vi "Wait For Stream Drain.vi"(8 "error in":errorcluster, 10 "timeout ms":i32=1000, 11 "events":refnum<queue>) -> (0 "error out":errorcluster, 3 "drained?":bool)   [LabVIEW 2020, in "MCP Server.lvlib"]
doc: "Waits until the events queue of a streamed tools/call is empty, polling every 20 ms, for at most timeout ms.\n\nWhile the client is connected, the IG HTTP Server sends one event per Next Segment call and asks for the next one straight away, so the queue empties within milliseconds. When the client has closed the stream, a chunk write fails, the server stops asking and nothing empties the queue any more: drained? stays FALSE. That is how a closed stream (the MCP cancellation signal over HTTP) is noticed. An invalid or released queue also gives FALSE."
uses:
  MCP Server.lvlib
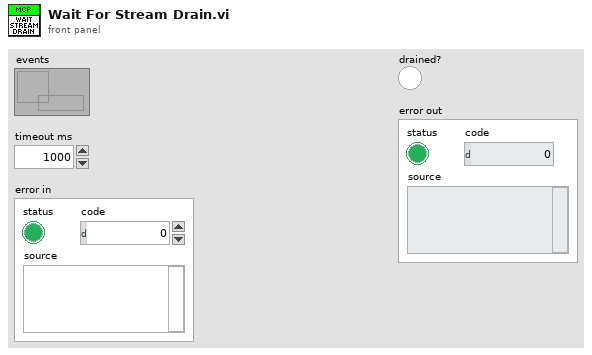
[diagram p1: front panel]
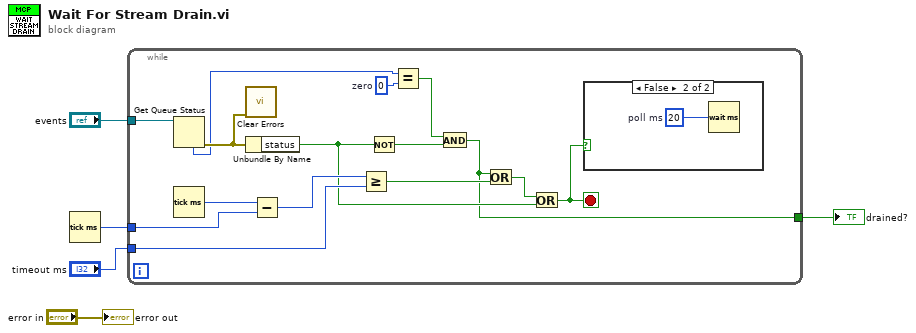
[diagram p0: block diagram]
diagram:
  n1 = Tick Count (ms)() -> (millisecond timer value=w4:u32)
  n2 = while {
    tunnel: "events" -> [w20]
    tunnel: w4 -> [w13]
    tunnel: "timeout ms" -> [w11]
    tunnel: [w6] -> w2
    stop <- w7 stop-if-true
    w17 = 0  # zero
    n3 = Get Queue Status(queue=w20) -> (error out=w19:errorcluster, # elements in queue=w18:i32)  [unwired: 2 in, 6 out]
    n4 = Tick Count (ms)() -> (millisecond timer value=w14:u32)
    n5 = call <vilib>:"Clear Errors.vi"("error in (no error)"=w19) -> ()  [unwired: 5 in, 2 out]
    n6 = Unbundle By Name(w19) -> ("status"=w8:bool)
    n7 = Subtract(x=w14, y=w13) -> (x-y=w12:u32)
    n8 = Greater Or Equal?(x=w12, y=w11) -> (x >= y?=w10:bool)
    n9 = Not(x=w8) -> (.not. x?=w15:bool)
    n10 = Equal?(x=w18, y=w17) -> (x = y?=w16:bool)
    n11 = And(x=w16, y=w15) -> (x .and. y?=w6:bool)
    n12 = Or(x=w6, y=w10) -> (x .or. y?=w9:bool)
    n13 = Or(x=w9, y=w8) -> (x .or. y?=w7:bool)
    n14 = case shown="False" w7 {
      frame True {
      }
      frame False {
        w21 = u32 20  # poll ms
        n15 = Wait (ms)(milliseconds to wait=w21) -> ()  [unwired: 1 out]
      }
    }
  }
  "drained?" <- w2
  "error out" <- "error in"
